vi "PRES+TEMP+REG V115.vi"() -> ()   [LabVIEW 2022 SP3]
uses:
  Enum/Enum 9.ctl
  Variables globales/Variable glob generale.vi
  Variables globales/Variables glob EUROTHERM.vi
panel:
  in  "Mails":bool
  in  "Logbook":bool
  in  "gestion reg EUROTHERM":bool caption="choix 2"
  in  "créer profil reg EUROTHERM":bool caption="choix 2"
  in  "Surveillance":bool
  in  "choix":bool
  in  "Visualisation":bool
  in  "Arrêt":bool
  in  "Lancer":bool
  # "acquisitions\ninstrumentation"
  # "ACQUISITIONS :"
  # "CONFIGURATION\nDES RÉGULATEURS :"
  # "Ce logiciel et les informations qu'il contient, sont la propriété de l’IAS et ne peuvent être diffusés sans l’autorisation de la Station d’étalonnage"
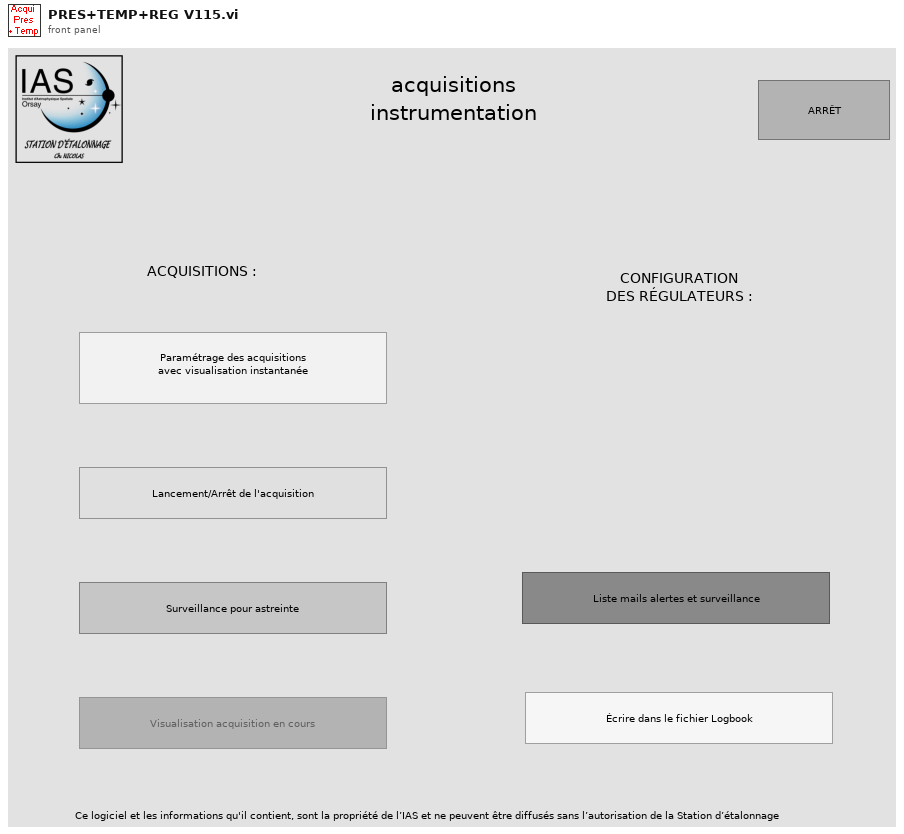
[diagram p1: front panel]
types:
  T1 = typedef "Enum 9.ctl" = enum16{"init var glog", "LUV ou NEPTUNE", "premier menu", "choix", "fermer"}
  T2 = enum8{"Enabled", "Disabled", "Disabled and Grayed Out"}
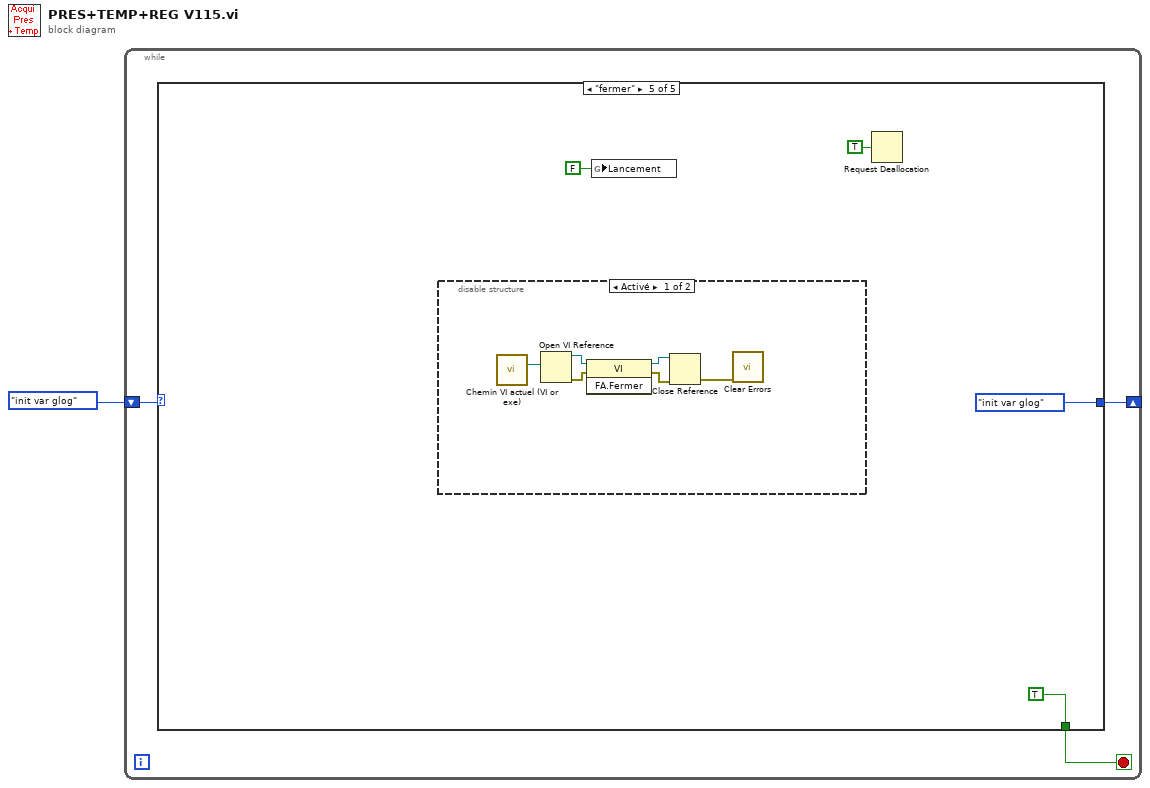
[diagram p0: block diagram]
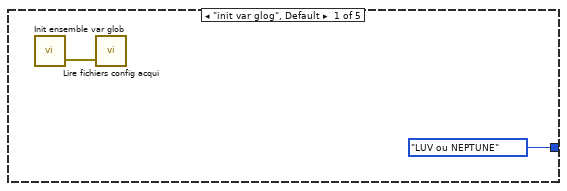
[diagram p2: hidden frame]
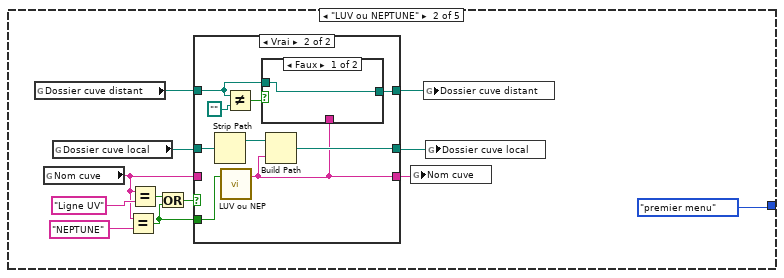
[diagram p3: hidden frame]
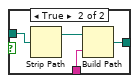
[diagram p5: hidden frame]
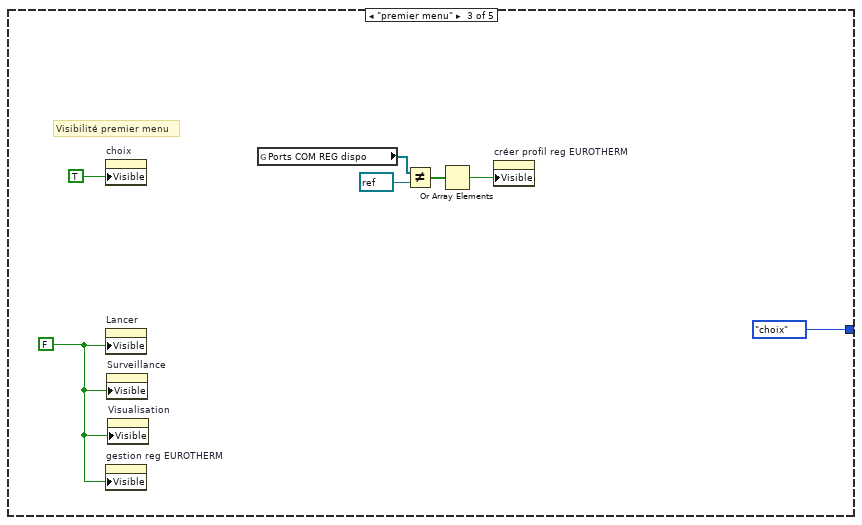
[diagram p6: hidden frame]
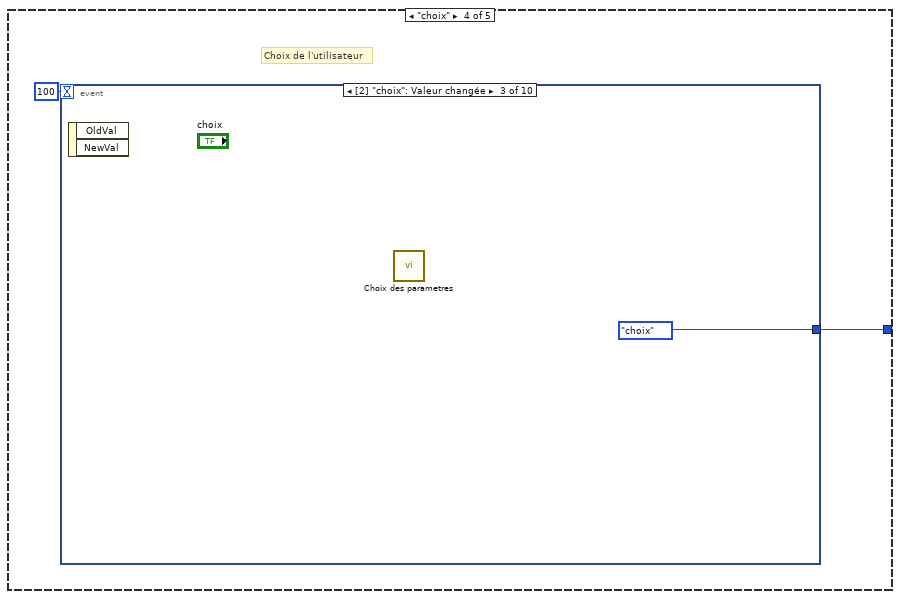
[diagram p7: hidden frame]
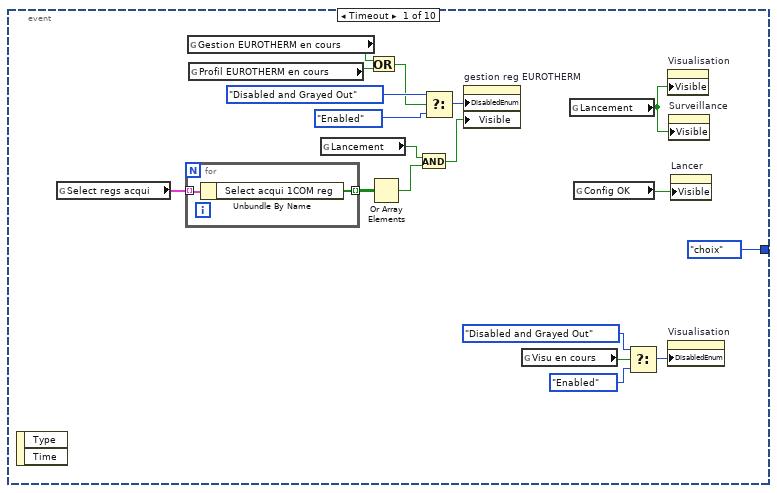
[diagram p8: hidden frame]
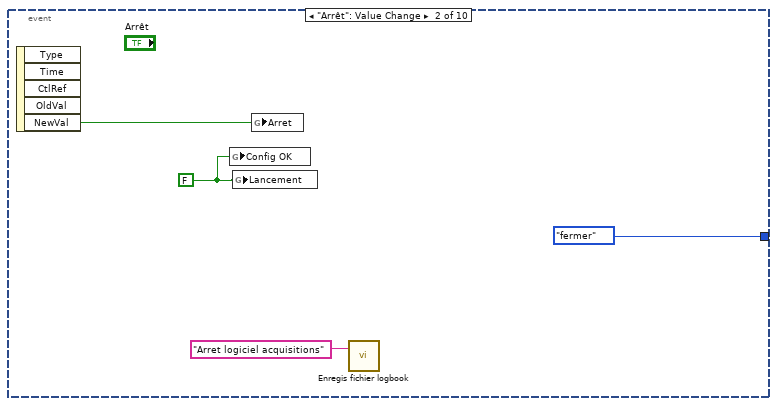
[diagram p9: hidden frame]
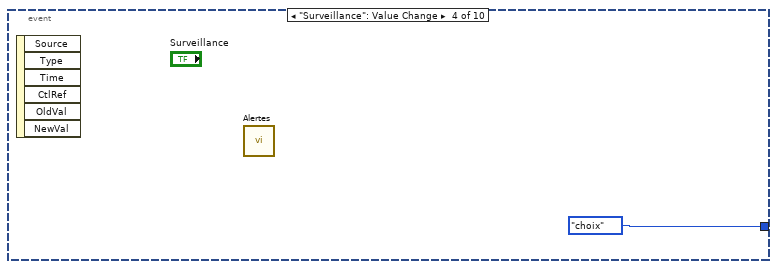
[diagram p10: hidden frame]
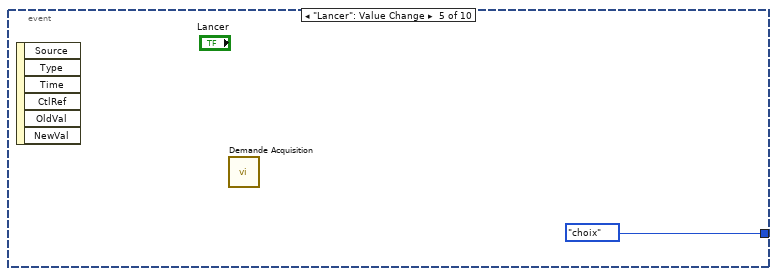
[diagram p11: hidden frame]
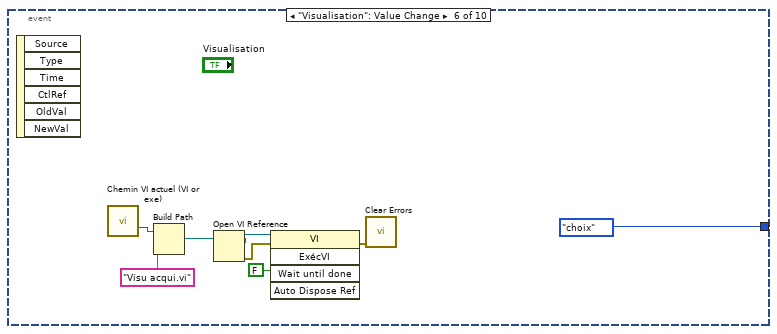
[diagram p12: hidden frame]
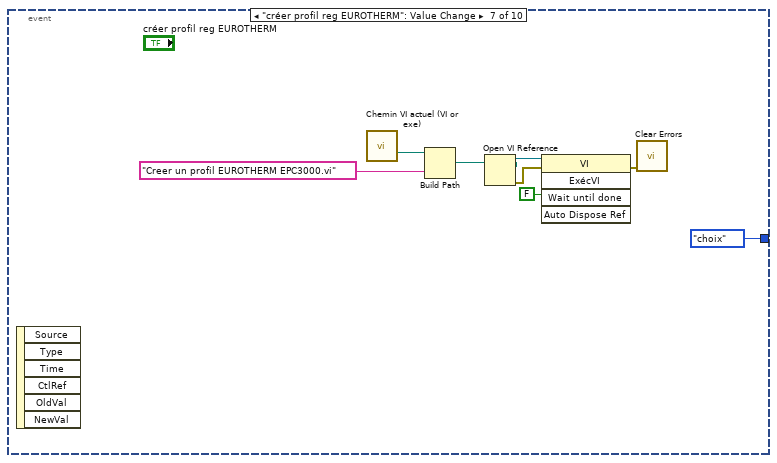
[diagram p13: hidden frame]
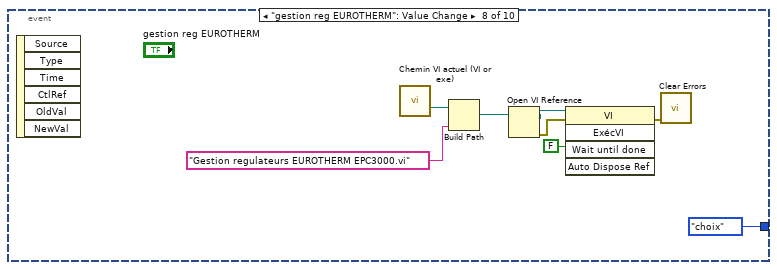
[diagram p14: hidden frame]
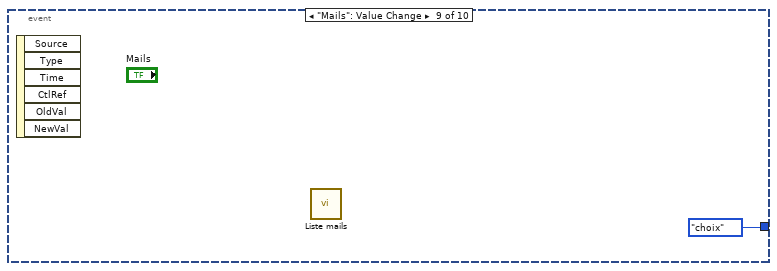
[diagram p15: hidden frame]
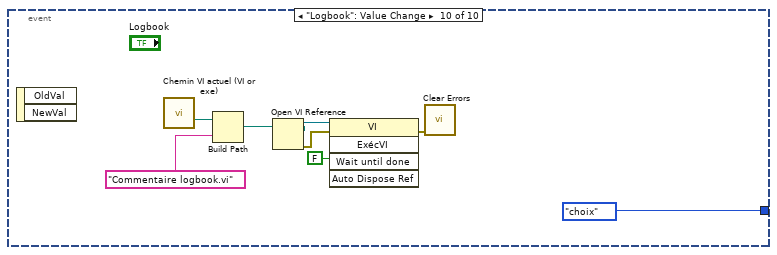
[diagram p16: hidden frame]
diagram:
  n1 = while {
    shift-right: [w3] -> _
    shift-left: Enum_9."init var glog" ("Énum") -> [w4]
    stop <- w2 stop-if-true
    n2 = case shown="\"fermer\"" w4 {
      tunnel: [Enum_9."LUV ou NEPTUNE" ("Énum") Enum_9."premier menu" ("Énum") Enum_9."choix" ("Énum") w43 Enum_9."init var glog" ("Énum")] -> w3
      tunnel: [_ _ _ _ TRUE] -> w2
      frame "init var glog", Default {
        n3 = call "Init ensemble var glob.vi"() -> ("error out"=w5:errorcluster)  [unwired: 3 in]
        n4 = call "Lire fichiers config acqui.vi"("error in (no error)"=w5) -> ()  [unwired: 2 in, 1 out]
      }
      frame "LUV ou NEPTUNE" {
        n5 = global read "Variable glob generale.vi" "Dossier cuve distant"() -> (w14:path)
        n6 = global read "Variable glob generale.vi" "Nom cuve"() -> (w12:string)
        n7 = global read "Variable glob generale.vi" "Dossier cuve local"() -> (w13:path)
        n8 = Equal?(x=w12, y="NEPTUNE") -> (x = y?=w8:bool)
        n9 = Equal?(x=w12, y="Ligne UV") -> (x = y?=w10:bool)
        n10 = Or(x=w10, y=w8) -> (x .or. y?=w9:bool)
        n11 = case shown="Vrai" w9 {
          tunnel: w12 -> [w21 _]
          tunnel: [w21 w23] -> w16
          tunnel: w13 -> [w20 w28]
          tunnel: w14 -> [w19 w22]
          tunnel: [w20 w29] -> w17
          tunnel: [w19 w30] -> w18
          tunnel: w8 -> [_ w26]
          frame False {
          }
          frame True {
            n12 = Strip Path(path=w28) -> (stripped path=w27:path)  [unwired: 1 out]
            n13 = call "LUV ou NEP.vi"("Booléen"=w26) -> ("Nom cuve"=w23:string)  [unwired: 2 in]
            n14 = Not Equal?(x=w22, y=path "") -> (x != y?=w24:bool)
            n15 = case shown="Faux" w24 {
              tunnel: [w31 w35] -> w30
              tunnel: w22 -> [w31 w33]
              tunnel: w23 -> [_ w34]
              frame False {
              }
              frame True {
                n16 = Strip Path(path=w33) -> (stripped path=w32:path)  [unwired: 1 out]
                n17 = Build Path(base path=w32, name or relative path=w34) -> (appended path=w35:path)
              }
            }
            n18 = Build Path(base path=w27, name or relative path=w23) -> (appended path=w29:path)
          }
        }
        n19 = global write "Variable glob generale.vi" "Nom cuve"(w16) -> ()
        n20 = global write "Variable glob generale.vi" "Dossier cuve distant"(w18) -> ()
        n21 = global write "Variable glob generale.vi" "Dossier cuve local"(w17) -> ()
      }
      frame "premier menu" {
        w38 = FALSE
        # "Visibilité premier menu"
        n22 = property on="choix" class="Bool"("Visible"=TRUE) -> ()  [unwired: 2 in, 2 out]
        n23 = property on="Lancer" class="Bool"("Visible"=w38) -> ()  [unwired: 2 in, 2 out]
        n24 = property on="gestion reg EUROTHERM" class="Bool"("Visible"=w38) -> ()  [unwired: 2 in, 2 out]
        n25 = property on="Surveillance" class="Bool"("Visible"=w38) -> ()  [unwired: 2 in, 2 out]
        n26 = property on="Visualisation" class="Bool"("Visible"=w38) -> ()  [unwired: 2 in, 2 out]
        n27 = global read "Variables glob EUROTHERM.vi" "Ports COM REG dispo"() -> (w39:refnum<visa-resource-name>[])
        n28 = Not Equal?(x=w39, y=refnum<visa-resource-name> refnum) -> (x != y?=w37:bool[])
        n29 = Or Array Elements(Boolean array=w37) -> (logical OR=w36:bool)
        n30 = property on="créer profil reg EUROTHERM" class="Bool"("Visible"=w36) -> ()  [unwired: 2 in, 2 out]
      }
      frame "choix" {
        # "Choix de l'utilisateur"
        n31 = event shown="[2] \"choix\": Valeur changée" {
          selector: _ -> [_ _ _ _ _ _ _ _ _ _]
          dyn-events: _ -> [_ _ _ _ _ _ _ _ _ _]
          timeout: 100 -> [_ _ _ _ _ _ _ _ _ _]
          tunnel: [Enum_9."choix" ("Énum") Enum_9."fermer" ("Énum") Enum_9."choix" ("Énum") Enum_9."choix" ("Énum") Enum_9."choix" ("Énum") Enum_9."choix" ("Énum") Enum_9."choix" ("Énum") Enum_9."choix" ("Énum") Enum_9."choix" ("Énum") Enum_9."choix" ("Énum")] -> w43
          event Timeout {
            n32 = event-data() -> ()  [unwired: 1 in, 2 out]
            n33 = global read "Variables glob EUROTHERM.vi" "Select regs acqui"() -> (w46:cluster{"Select acqui 1COM reg":bool[]}[])
            n34 = for {
              tunnel: w46 -> [w64] mode=indexing
              tunnel: [w63] -> w45 mode=indexing
              n35 = Unbundle By Name(w64) -> ("Select acqui 1COM reg"=w63:bool[])
            }
            n36 = global read "Variable glob generale.vi" "Gestion EUROTHERM en cours"() -> (w53:bool)
            n37 = global read "Variable glob generale.vi" "Profil EUROTHERM en cours"() -> (w52:bool)
            n38 = global read "Variable glob generale.vi" "Lancement"() -> (w49:bool)
            n39 = Or(x=w53, y=w52) -> (x .or. y?=w51:bool)
            n40 = Or Array Elements(Boolean array=w45) -> (logical OR=w47:bool)
            n41 = And(x=w49, y=w47) -> (x .and. y?=w48:bool)
            n42 = Select(t=T2."Disabled and Grayed Out" ("Désactivé"), s=w51, f=T2."Enabled" ("Désactivé")) -> (s? t:f=w56:T2)
            n43 = property on="gestion reg EUROTHERM" class="Bool"("DisabledEnum"=w56, "Visible"=w48) -> ()  [unwired: 2 in, 2 out]
            n44 = global read "Variable glob generale.vi" "Visu en cours"() -> (w58:bool)
            n45 = global read "Variable glob generale.vi" "Lancement"() -> (w61:bool)
            n46 = global read "Variable glob generale.vi" "Config OK"() -> (w62:bool)
            n47 = Select(t=T2."Disabled and Grayed Out" ("Désactivé"), s=w58, f=T2."Enabled" ("Désactivé")) -> (s? t:f=w60:T2)
            n48 = property on="Visualisation" class="Bool"("Visible"=w61) -> ()  [unwired: 2 in, 2 out]
            n49 = property on="Visualisation" class="Bool"("DisabledEnum"=w60) -> ()  [unwired: 2 in, 2 out]
            n50 = property on="Surveillance" class="Bool"("Visible"=w61) -> ()  [unwired: 2 in, 2 out]
            n51 = property on="Lancer" class="Bool"("Visible"=w62) -> ()  [unwired: 2 in, 2 out]
          }
          event "Arrêt": Value Change {
            w68 = FALSE ("Lancement")
            n52 = event-data() -> ("NewVal"=w67:bool)  [unwired: 1 in, 4 out]
            n53 = global write "Variable glob generale.vi" "Config OK"(w68) -> ()
            n54 = global write "Variable glob generale.vi" "Lancement"(w68) -> ()
            n55 = global write "Variable glob generale.vi" "Arret"(w67) -> ()
            n56 = call "Enregis fichier logbook.vi"("Chaîne"="Arret logiciel acquisitions") -> ()  [unwired: 2 in, 1 out]
          }
          event "choix": Value Change {
            n57 = event-data() -> ()  [unwired: 1 in, 2 out]
            n58 = call "Choix des parametres.vi"() -> ()  [unwired: 4 in]
          }
          event "Surveillance": Value Change {
            n59 = event-data() -> ()  [unwired: 1 in, 6 out]
            n60 = call "Alertes.vi"() -> ()  [unwired: 4 in]
          }
          event "Lancer": Value Change {
            n61 = event-data() -> ()  [unwired: 1 in, 6 out]
            n62 = call "Demande Acquisition.vi"() -> ()  [unwired: 4 in]
          }
          event "Visualisation": Value Change {
            n63 = event-data() -> ()  [unwired: 1 in, 6 out]
            n64 = call "Chemin VI actuel (VI or exe).vi"() -> ("VI or executable installation directory"=w73:path)  [unwired: 14 in, 1 out]
            n65 = Build Path(base path=w73, name or relative path="Visu acqui.vi" ("nom ou chemin relatif")) -> (appended path=w78:path)
            n66 = Open VI Reference(vi path=w78) -> (vi reference=w76:refnum<vi>, error out=w75:errorcluster)  [unwired: 5 in]
            n67 = invoke class="VI" method="ExécVI"(reference=w76, error in=w75, "Wait until done"=FALSE ("Attendre la fin")) -> (error out=w74:errorcluster)  [unwired: 2 in, 4 out]
            n68 = call <vilib>:"Clear Errors.vi"("error in (no error)"=w74) -> ()  [unwired: 5 in, 2 out]
          }
          event "créer profil reg EUROTHERM": Value Change {
            n69 = event-data() -> ()  [unwired: 1 in, 6 out]
            n70 = call "Chemin VI actuel (VI or exe).vi"() -> ("VI or executable installation directory"=w82:path)  [unwired: 14 in, 1 out]
            n71 = Build Path(base path=w82, name or relative path="Creer un profil EUROTHERM EPC3000.vi" ("nom ou chemin relatif")) -> (appended path=w87:path)
            n72 = Open VI Reference(vi path=w87) -> (vi reference=w85:refnum<vi>, error out=w84:errorcluster)  [unwired: 5 in]
            n73 = invoke class="VI" method="ExécVI"(reference=w85, error in=w84, "Wait until done"=FALSE ("Attendre la fin")) -> (error out=w83:errorcluster)  [unwired: 2 in, 4 out]
            n74 = call <vilib>:"Clear Errors.vi"("error in (no error)"=w83) -> ()  [unwired: 5 in, 2 out]
          }
          event "gestion reg EUROTHERM": Value Change {
            n75 = event-data() -> ()  [unwired: 1 in, 6 out]
            n76 = call "Chemin VI actuel (VI or exe).vi"() -> ("VI or executable installation directory"=w90:path)  [unwired: 14 in, 1 out]
            n77 = Build Path(base path=w90, name or relative path="Gestion regulateurs EUROTHERM EPC3000.vi" ("nom ou chemin relatif")) -> (appended path=w95:path)
            n78 = Open VI Reference(vi path=w95) -> (vi reference=w93:refnum<vi>, error out=w92:errorcluster)  [unwired: 5 in]
            n79 = invoke class="VI" method="ExécVI"(reference=w93, error in=w92, "Wait until done"=FALSE ("Attendre la fin")) -> (error out=w91:errorcluster)  [unwired: 2 in, 4 out]
            n80 = call <vilib>:"Clear Errors.vi"("error in (no error)"=w91) -> ()  [unwired: 5 in, 2 out]
          }
          event "Mails": Value Change {
            n81 = event-data() -> ()  [unwired: 1 in, 6 out]
            n82 = call "Liste mails.vi"() -> ()  [unwired: 12 in]
          }
          event "Logbook": Value Change {
            n83 = event-data() -> ()  [unwired: 1 in, 2 out]
            n84 = call "Chemin VI actuel (VI or exe).vi"() -> ("VI or executable installation directory"=w98:path)  [unwired: 14 in, 1 out]
            n85 = Build Path(base path=w98, name or relative path="Commentaire logbook.vi" ("nom ou chemin relatif")) -> (appended path=w103:path)
            n86 = Open VI Reference(vi path=w103) -> (vi reference=w101:refnum<vi>, error out=w100:errorcluster)  [unwired: 5 in]
            n87 = invoke class="VI" method="ExécVI"(reference=w101, error in=w100, "Wait until done"=FALSE ("Attendre la fin")) -> (error out=w99:errorcluster)  [unwired: 2 in, 4 out]
            n88 = call <vilib>:"Clear Errors.vi"("error in (no error)"=w99) -> ()  [unwired: 5 in, 2 out]
          }
        }
      }
      frame "fermer" {
        n89 = disable-structure shown="Activé" {
          frame Enabled {
            n90 = call "Chemin VI actuel (VI or exe).vi"() -> ("Full Path to VI or executable"=w114:path)  [unwired: 14 in, 1 out]
            n91 = Open VI Reference(vi path=w114) -> (vi reference=w113:refnum<vi>, error out=w112:errorcluster)  [unwired: 5 in]
            n92 = invoke class="VI" method="FA.Fermer"(reference=w113, error in=w112) -> (reference out=w110:refnum<vi>, error out=w111:errorcluster)  [unwired: 1 in, 1 out]
            n93 = Close Reference(reference=w110, error in (no error)=w111) -> (error out=w109:errorcluster)
            n94 = call <vilib>:"Clear Errors.vi"("error in (no error)"=w109) -> ()  [unwired: 5 in, 2 out]
          }
          frame Disabled {
          }
        }
        n95 = global write "Variable glob generale.vi" "Lancement"(FALSE) -> ()
        n96 = Request Deallocation(TRUE ("flag")) -> ()
      }
    }
  }
